vi "FuncVI_Sub - Dialog Box.vi"(4 "data":string, 5 "message":string) -> (0 "True ?":bool, 2 "string out":string)   [LabVIEW 2021]
doc: "::: CalcExpress Toolkit :::\nCopyright (c) 2000-2026 Konstantin Shifershteyn. All rights reserved."
panel:
  in  "cancel":bool
  in  "ok":bool
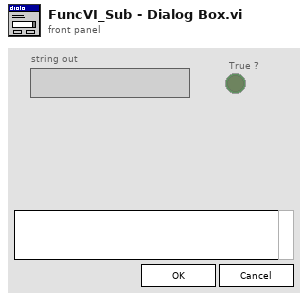
[diagram p1: front panel]
types:
  T1 = typedef "eventvkey.ctl" = enum16{"ASCII", "Enter", "Return", "Shift", "Ctrl", "Alt", "Cmd", "Opt", "Caps", "NumLock", "Clear", "Break", "Up", "Down", "Left", "Right", "Insert", "Delete", "Home", "End", "PageUp", "PageDown", "Escape", "Help", "Pause", "ScrollLock", "F1", "F2", "F3", "F4", "F5", "F6", "F7", "F8", "F9", "F10", "F11", "F12", "F13", "F14", "F15", "F16", "F17", "F18", "F19", "F20", "F21", "F22", "F23", "F24", "Play", "VolumeUp", "VolumeDown", "Mute", "Two Byte Char"}
  T2 = cluster{"Shift":bool, "Ctrl":bool, "Alt":bool, "Cmd":bool, "Opt":bool}
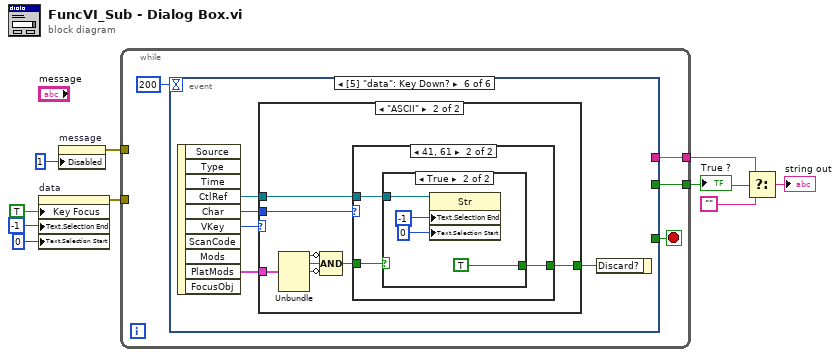
[diagram p0: block diagram]
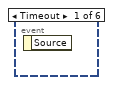
[diagram p2: hidden frame]
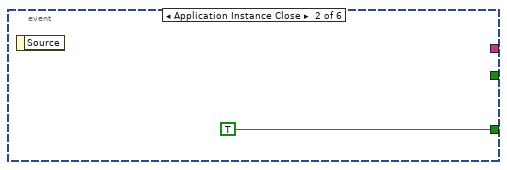
[diagram p3: hidden frame]
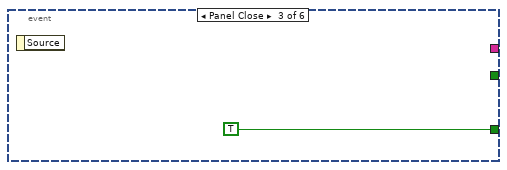
[diagram p4: hidden frame]
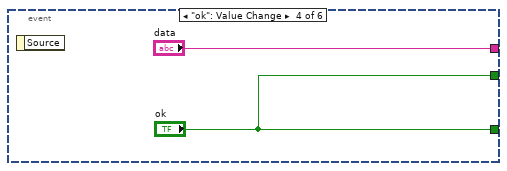
[diagram p5: hidden frame]
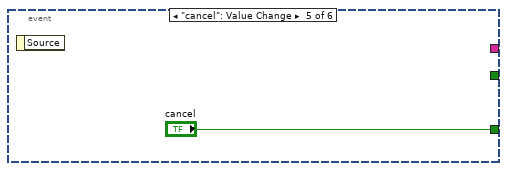
[diagram p6: hidden frame]
diagram:
  n1 = property on="data" class="Str"("Key Focus"=TRUE, "Text.Selection End"=-1, "Text.Selection Start"=u32 0 ("Text.Selection:Start")) -> (error out=w3:errorcluster)  [unwired: 2 in, 1 out]
  n2 = property on="message" class="Str"("Disabled"=u8 1) -> (error out=w4:errorcluster)  [unwired: 2 in, 1 out]
  n3 = while {
    tunnel: [w12] -> w6
    tunnel: [w11] -> w5
    tunnel: w4 -> [_]
    tunnel: w3 -> [_]
    stop <- w13 stop-if-true
    n4 = event shown="[5] \"data\": Key Down?" {
      selector: _ -> [_ _ _ _ _ _]
      dyn-events: _ -> [_ _ _ _ _ _]
      timeout: 200 -> [_ _ _ _ _ _]
      tunnel: [_ TRUE TRUE "ok" "cancel" _] -> w13
      tunnel: [_ _ _ "ok" _ _] -> w12
      tunnel: [_ _ _ "data" _ _] -> w11
      event Timeout {
        n5 = event-data() -> ()  [unwired: 1 in, 1 out]
      }
      event Application Instance Close {
        n6 = event-data() -> ()  [unwired: 1 in, 1 out]
      }
      event Panel Close {
        n7 = event-data() -> ()  [unwired: 1 in, 1 out]
      }
      event "ok": Value Change {
        n8 = event-data() -> ()  [unwired: 1 in, 1 out]
      }
      event "cancel": Value Change {
        n9 = event-data() -> ()  [unwired: 1 in, 1 out]
      }
      event "data": Key Down? {
        n10 = event-data() -> ("CtlRef"=w21:refnum<vi>, "Char"=w22:i16, "VKey"=w24:T1, "PlatMods"=w23:T2)  [unwired: 1 in, 6 out]
        n11 = case shown="\"ASCII\"" w24 {
          tunnel: w23 -> [_ w32]
          tunnel: w22 -> [_ w28]
          tunnel: w21 -> [_ w27]
          tunnel: [_ w25] -> w20
          frame Default {
          }
          frame "ASCII" {
            n12 = Unbundle(w32) -> ("Shift"=w31:bool, "Ctrl"=w30:bool, "Alt"=w29:bool)  [unwired: 2 out]
            n13 = Compound Arithmetic op=AND(invert w31, w30, invert w29) -> (w26:bool)
            n14 = case shown="41, 61" w28 {
              tunnel: w27 -> [_ w35]
              tunnel: w26 -> [_ w34]
              tunnel: [_ w33] -> w25
              frame Default {
              }
              frame 65, 97 {
                n15 = case shown="True" w34 {
                  tunnel: w35 -> [_ w39]
                  tunnel: [_ TRUE] -> w33
                  frame False {
                  }
                  frame True {
                    n16 = property class="Str"(reference=w39, "Text.Selection End"=-1, "Text.Selection Start"=u32 0 ("Text.Selection:Start")) -> ()  [unwired: 1 in, 2 out]
                  }
                }
              }
            }
          }
        }
        n17 = event-data("Discard?"=w20) -> ()  [unwired: 1 in, 1 out]
      }
    }
  }
  "True ?" <- w6
  n18 = Select(t=w5, s=w6, f="") -> (s? t:f=→"string out":string)
